vi "Bollen-numb.vi"(10 "布尔 2":bool, 11 "布尔":bool) -> (3 "数字":u32)   [LabVIEW 2025]
panel:
  # "4个情况代表4个数字\n2-3-6-7"
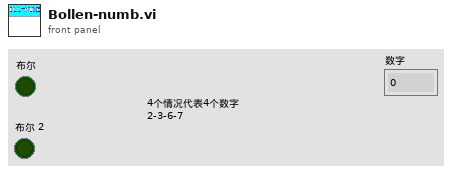
[diagram p1: front panel]
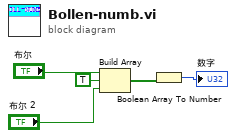
[diagram p0: block diagram]
diagram:
  n1 = Build Array("布尔", TRUE ("元素"), "布尔 2") -> (w3:bool[])
  n2 = Boolean Array To Number(Boolean array=w3) -> (number=→"数字":u32)
